vi "New File Handler.vi"(6 "file name format (\"logfile_%<%Y-%m-%d_%H-%M-%S>T.log\")":string="logfile_%<%Y-%m-%d_%H-%M-%S>T.log", 7 "max file size [MB](50)":dbl=50.0, 8 "error in":errorcluster, 9 "cleanup age [days](30)":dbl=30.0, 10 "formatter (JSON)":refnum<class "Formatter.lvclass">, 11 "log directory (<app dir>/logs)":path) -> (0 "error out":errorcluster, 2 "events":T1, 3 "file handler":refnum<class "File Handler.lvclass">)   [LabVIEW 2018, in "GLog.lvlib" / "File Handler.lvclass"]
doc: "Creates a new Handler which writes log records to a file."
uses:
  File Handler.lvclass
  extension/formatter_interface/Formatter.lvclass
  Events.ctl
  File Update Event.ctl
  RolloverTrigger.Size/RolloverTrigger.Size.lvclass
  C:/Users/Colin/Documents/software_projects/labview/glog/src/api/configuration/handlers/file_handler/RolloverTrigger/RolloverTrigger.lvclass
  CleanupFilter.LastMod/CleanupFilter.LastMod.lvclass
  C:/Users/Colin/Documents/software_projects/labview/glog/src/api/configuration/handlers/file_handler/CleanupFilter/CleanupFilter.lvclass
panel:
  # "Connector Pane"
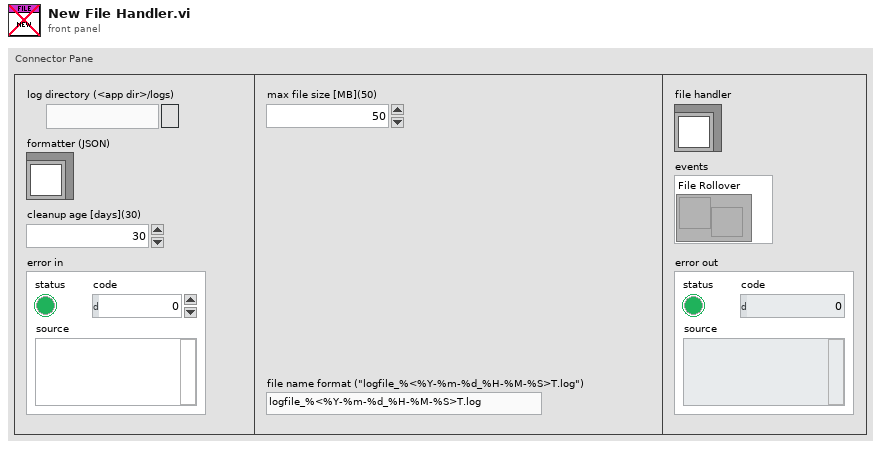
[diagram p1: front panel]
types:
  T1 = typedef "GLog.lvlib/File Handler.lvclass/Events.ctl" = cluster{"File Rollover":refnum<user-event>}
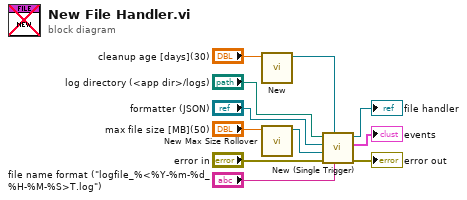
[diagram p0: block diagram]
diagram:
  n1 = call "New.vi"("age limit [days](30)"="cleanup age [days](30)") -> ("Cleanup Filter"=w2:refnum<class "CleanupFilter.LastMod.lvclass">)  [unwired: 10 in]
  n2 = call "New Max Size Rollover.vi"("max file size [MB](50)"="max file size [MB](50)") -> ("size trigger"=w4:refnum<class "RolloverTrigger.Size.lvclass">)  [unwired: 10 in]
  n3 = call "New (Single Trigger).vi"("file name format (\"logfile_%<%Y-%m-%d_%H-%M-%S>T.log\")"="file name format (\"logfile_%<%Y-%m-%d_%H-%M-%S>T.log\")", "cleanup filter (never)"=w2, "error in"="error in", "rollover trigger (50 MB)"=w4, "formatter (JSON)"="formatter (JSON)", "log directory (<app dir>/logs)"="log directory (<app dir>/logs)") -> ("error out"=→"error out":errorcluster, "events"=→"events":T1, "file handler"=→"file handler":refnum<class "File Handler.lvclass">)  [unwired: 3 in]
